vi "SetVarVal.vi"(8 "error in (no error)":errorcluster, 9 "varValue":dbl, 10 "varName":string, 11 "muExpr in":refnum<class "mupExpr.lvclass">) -> (0 "error out":errorcluster, 3 "muExpr out":refnum<class "mupExpr.lvclass">)   [LabVIEW 2018, in "mupExpr.lvclass"]
uses:
  mupExpr.lvclass
  mupExpr.lvclass/mupExpr.ctl
  <vilib>/Utility/error.llb/Error Cluster From Error Code.vi
  <vilib>/ErrorRing/Error Ring.xnode
  mupLib/mupLib.lvlib
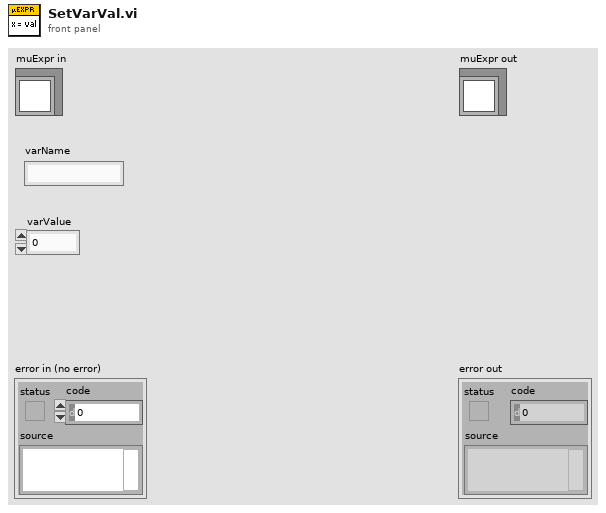
[diagram p1: front panel]
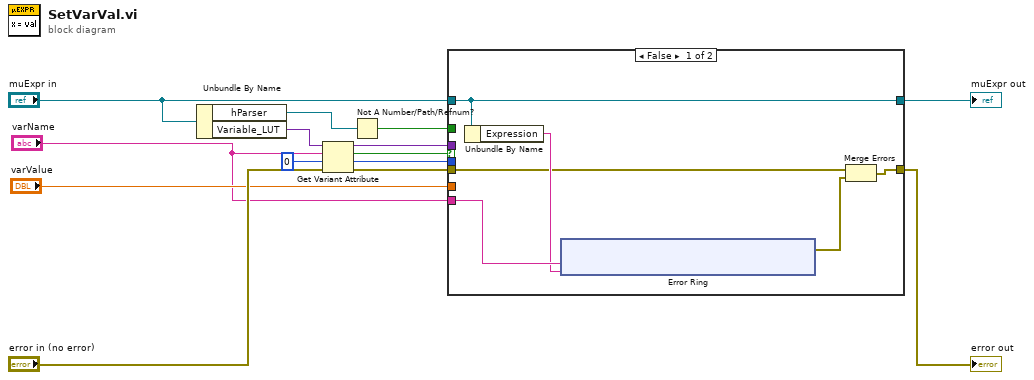
[diagram p0: block diagram]
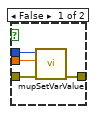
[diagram p3: hidden frame]
diagram:
  n1 = Unbundle By Name("muExpr in") -> ("hParser"=w3:refnum<data-value>, "Variable_LUT"=w8:variant)
  n2 = Get Variant Attribute(Variant=w8, name="varName", default value (empty Variant)=u64 0 ("pd"), error in="error in (no error)") -> (duplicate Variant=w4:variant, found=w2:bool, value=w5:u64, error out=w7:errorcluster)
  n3 = Not A Number/Path/Refnum?(number/path/refnum=w3) -> (NaN/Path/Refnum?=w1:bool)
  n4 = case shown="False" w2 {
    tunnel: w7 -> [w16 w33]
    tunnel: "varValue" -> [_ w31]
    tunnel: w5 -> [_ w30]
    tunnel: [w17 w32] -> w13
    tunnel: "varName" -> [w19 _]
    tunnel: "muExpr in" -> [w20 w34]
    tunnel: w4 -> [_ _]
    tunnel: [w20 w34] -> w11
    tunnel: w1 -> [_ w29]
    frame False {
      n5 = Unbundle By Name(w20) -> ("Expression"=w18:string)
      n6 = xnode "Error Ring"("parameter 0"=w19, "parameter 1"=w18) -> ("error out"=w15:errorcluster)
      n7 = Merge Errors(w16, w15) -> (w17:errorcluster)
    }
    frame True {
      n8 = case shown="True" w29 {
        tunnel: w33 -> [w38 w39]
        tunnel: [w37 w39] -> w32
        tunnel: w31 -> [w36 _]
        tunnel: w30 -> [w35 _]
        frame False {
          n9 = call "mupSetVarValue.vi"("error in (no error)"=w38, "varValue"=w36, "varAddr in"=w35) -> ("error out"=w37:errorcluster)  [unwired: 7 in, 1 out]
        }
        frame True {
        }
      }
    }
  }
  "error out" <- w13
  "muExpr out" <- w11
